vi "VHist - generate numeric sequence.vi"(5 "inclusive (T)":bool=TRUE, 7 "step":dbl format="%.2f", 8 "final value":dbl format="%.2f", 9 "initial value":dbl format="%.2f") -> (0 "error":bool, 3 "array out":dbl[](array[numeric]) format="%.2f")   [LabVIEW 2021]
doc: "::: CalcExpress Toolkit :::\nCopyright (c) 2000-2026 Konstantin Shifershteyn. All rights reserved."
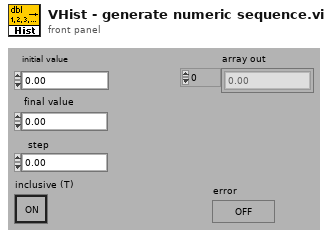
[diagram p1: front panel]
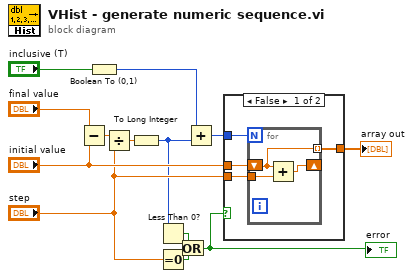
[diagram p0: block diagram]
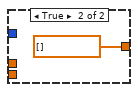
[diagram p2: hidden frame]
diagram:
  n1 = Subtract(x="final value", y="initial value") -> (x-y=w13:dbl)
  n2 = Boolean To (0,1)(Boolean="inclusive (T)") -> (0, 1=w2:i16)
  n3 = Divide(x=w13, y="step") -> (x/y=w4:dbl)
  n4 = To Long Integer(number=w4) -> (32bit integer=w5:i32)
  n5 = Less Than 0?(x=w5) -> (x < 0?=w12:bool)
  n6 = Equal To 0?(x="step") -> (x = 0?=w11:bool)
  n7 = Or(x=w12, y=w11) -> (x .or. y?=w7:bool)
  "error" <- w7
  n8 = Add(x=w2, y=w5) -> (x+y=w6:i32)
  n9 = case shown="False" w7 {
    tunnel: w6 -> [w17 _]
    tunnel: "initial value" -> [w16 _]
    tunnel: [w15 dbl[] []] -> w1
    tunnel: "step" -> [w14 _]
    frame False {
      n10 = for {
        N: w17 -> [_]
        shift-right: [w20] -> _
        shift-left: w16 -> [w18]
        tunnel: [w18] -> w15 mode=indexing
        tunnel: w14 -> [w19]
        n11 = Add(x=w18, y=w19) -> (x+y=w20:dbl)
      }
    }
    frame True {
    }
  }
  "array out" <- w1
